vi "Add Licence Information.vi"() -> ()   [LabVIEW 2019]
doc: "Running this VI from within a project will append a license text to the description of all source (below /src/ catalogue) VI's in that project."
panel:
  out "Files which needed to be modified":string[](array[string])
  in  "Copyright Notice":string="Copyright (c) 2025 KoRElibs.com"
  out "Total Files":dbl
  in  "License Text":string="SPDX-License-Identifier: EUPL-1.2\n\nThis VI is licensed under the European Union Public License (EUPL) Version 1.2. You may use this VI unmodified in proprietary works. If you distribute a modified version of this file, the modified file must be released under the EUPL-1.2. Full license: https://joinup.ec.europa.eu/asset/eupl/eupl/1.2/"
  out "Updates":i32
  out "Status":string
  out "Progress":dbl(slide) scale=0.0..1.0
  # "Running this VI will append the below copyright notice and license text to the description of all source (below /src/ catalogue) VI's in this project. If the Copyright Notice is allready included the license information is updated if necessary."
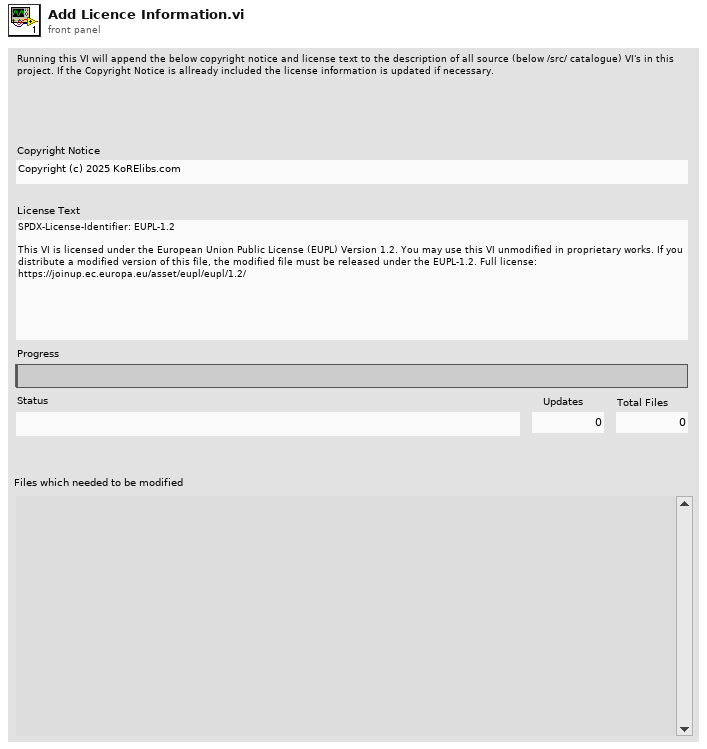
[diagram p1: front panel]
types:
  T1 = enum32{"Invalid", "Standard", "Closed", "Hidden", "Minimized", "Maximized"}
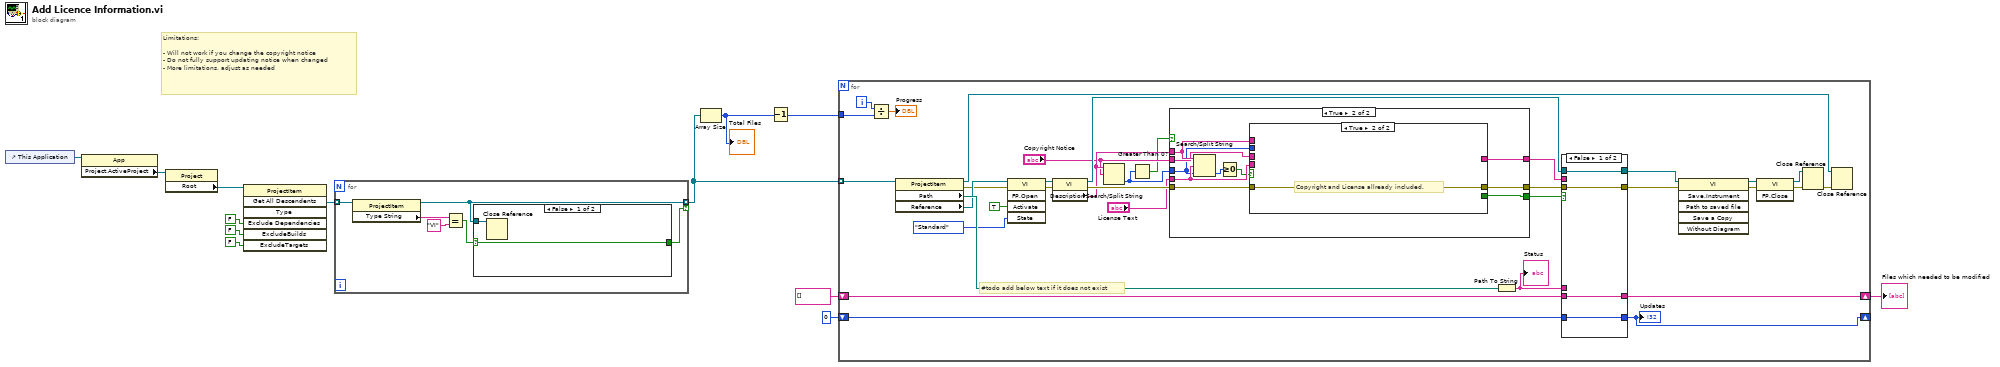
[diagram p0: block diagram]
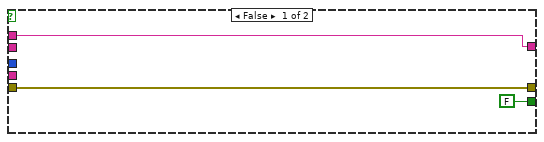
[diagram p2: hidden frame]
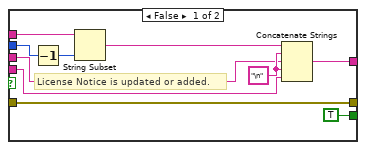
[diagram p3: hidden frame]
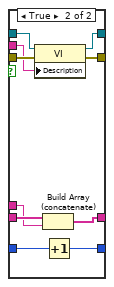
[diagram p4: hidden frame]
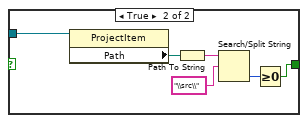
[diagram p5: hidden frame]
diagram:
  # "Limitations: \n\n- Will not work if you change the copyright notice\n- Do not fully support updating notice when changed\n- More limitations, adjust as needed"
  n1 = control-ref of="This Application"() -> (w13:refnum<vi>)
  n2 = property class="App"(reference=w13) -> ("Project.ActiveProject"=w12:refnum<vi>)  [unwired: 1 in, 2 out]
  n3 = property class="Project"(reference=w12) -> ("Root"=w11:refnum<vi>)  [unwired: 1 in, 2 out]
  n4 = invoke class="ProjectItem" method="Get All Descendents"(reference=w11, "Exclude Dependencies"=FALSE ("ExcludeDependencies"), "ExcludeBuilds"=FALSE, "ExcludeTargets"=FALSE) -> ("All Descendents"=w7:refnum<vi>[])  [unwired: 3 in, 6 out]
  n5 = for {
    tunnel: w7 -> [w19] mode=indexing
    tunnel: [w16] -> w6 mode=indexing if=w14
    n6 = property class="ProjectItem"(reference=w19) -> (reference out=w16:refnum<vi>, "Type String"=w17:string)  [unwired: 1 in, 1 out]
    n7 = Equal?(x=w17, y="VI") -> (x = y?=w15:bool)
    n8 = case shown="False" w15 {
      selector: w15 -> [w20 _]
      tunnel: w16 -> [w21 w27]
      tunnel: [w20 w22] -> w14
      frame False {
        n9 = Close Reference(reference=w21) -> ()  [unwired: 1 in, 1 out]
      }
      frame True {
        n10 = property class="ProjectItem"(reference=w27) -> ("Path"=w26:path)  [unwired: 1 in, 2 out]
        n11 = Path To String(path=w26) -> (string=w25:string)
        n12 = Search/Split String(string=w25, search string/char (-)="\\src\\") -> (offset of match=w23:i32)  [unwired: 1 in, 2 out]
        n13 = Greater Or Equal To 0?(x=w23) -> (x >= 0?=w22:bool)
      }
    }
  }
  n14 = Array Size(array=w6) -> (size(s)=w5:i32)
  "Total Files" <- w5
  n15 = Decrement(x=w5) -> (x-1=w4:i32)
  n16 = for {
    tunnel: w6 -> [w61] mode=indexing
    tunnel: w4 -> [w58]
    shift-right: [w50] -> _
    shift-left: 0 -> [w49]
    shift-right: [w46] -> w1
    shift-left: string[] [] -> [w48]
    i -> [w57]
    # "#todo add below text if it does not exist"
    n17 = Divide(x=w57, y=w58) -> (x/y=→"Progress":dbl)
    n18 = property class="ProjectItem"(reference=w61) -> (reference out=w60:refnum<vi>, error out=w39:errorcluster, "Path"=w56:path, "Reference"=w41:refnum<vi>)  [unwired: 1 in]
    n19 = invoke class="VI" method="FP.Open"(reference=w41, error in=w39, "Activate"=TRUE ("Activate?"), "State"=T1."Standard") -> (reference out=w40:refnum<vi>, error out=w38:errorcluster)  [unwired: 1 in, 3 out]
    n20 = property class="VI"(reference=w40, error in=w38) -> (reference out=w45:refnum<vi>, error out=w55:errorcluster, "Description"=w43:string)
    n21 = Search/Split String(string=w43, search string/char (-)="Copyright Notice") -> (offset of match=w29:i32)  [unwired: 1 in, 2 out]
    n22 = Greater Than 0?(x=w29) -> (x > 0?=w28:bool)
    n23 = case shown="True" w28 {
      tunnel: w55 -> [w63 w74]
      tunnel: [FALSE w73] -> w53
      tunnel: [w63 w72] -> w52
      tunnel: [w62 w71] -> w51
      tunnel: "License Text" -> [_ w70]
      tunnel: w43 -> [w62 w69]
      tunnel: "Copyright Notice" -> [_ w68]
      tunnel: w29 -> [_ w65]
      frame False {
      }
      frame True {
        n24 = Search/Split String(string=w69, search string/char (-)=w70, offset (0)=w65) -> (offset of match=w67:i32)  [unwired: 2 out]
        n25 = Greater Or Equal To 0?(x=w67) -> (x >= 0?=w66:bool)
        n26 = case shown="True" w66 {
          tunnel: [w81 w85] -> w72
          tunnel: w74 -> [w81 w85]
          tunnel: w65 -> [w84 _]
          tunnel: [TRUE _] -> w73
          tunnel: [w80 _] -> w71
          tunnel: w69 -> [w79 _]
          tunnel: w70 -> [w77 _]
          tunnel: w68 -> [w75 _]
          frame False {
            w76 = "\n" ("string")
            # "License Notice is updated or added."
            n27 = Decrement(x=w84) -> (x-1=w78:i32)
            n28 = String Subset(string=w79, length (rest)=w78) -> (substring=w83:string)  [unwired: 1 in]
            n29 = Concatenate Strings(w83, w76, w75, w76, w77) -> (w80:string)
          }
          frame True {
            # "Copyright and License allready included."
          }
        }
      }
    }
    n30 = Path To String(path=w56) -> (string=w47:string)
    "Status" <- w47
    n31 = case shown="False" w53 {
      tunnel: w45 -> [w89 w99]
      tunnel: w52 -> [w88 w98]
      tunnel: [w89 w97] -> w35
      tunnel: [w88 w96] -> w34
      tunnel: w51 -> [_ w95]
      tunnel: w49 -> [w87 w94]
      tunnel: [w87 w93] -> w50
      tunnel: w48 -> [w86 w92]
      tunnel: w47 -> [_ w90]
      tunnel: [w86 w91] -> w46
      frame False {
      }
      frame True {
        n32 = property class="VI"(reference=w99, error in=w98, "Description"=w95) -> (reference out=w97:refnum<vi>, error out=w96:errorcluster)
        n33 = Build Array (concatenate)(w92, w90) -> (w91:string[])
        n34 = Increment(x=w94) -> (x+1=w93:i32)
      }
    }
    "Updates" <- w50
    n35 = invoke class="VI" method="Save.Instrument"(reference=w35, error in=w34) -> (reference out=w33:refnum<vi>, error out=w31:errorcluster)  [unwired: 4 in, 4 out]
    n36 = invoke class="VI" method="FP.Close"(reference=w33, error in=w31) -> (reference out=w32:refnum<vi>, error out=w30:errorcluster)  [unwired: 1 in, 1 out]
    n37 = Close Reference(reference=w32, error in (no error)=w30) -> (error out=w54:errorcluster)
    n38 = Close Reference(reference=w60, error in (no error)=w54) -> ()  [unwired: 1 out]
  }
  "Files which needed to be modified" <- w1
